vi "CIVI Read Frequency.vi"(11 "VISA Resource Name":refnum<visa-resource-name>="TCPIP0::127.0.0.1::5025::SOCKET") -> (0 "error out":errorcluster, 3 "Frequency (Hz)":i32)   [LabVIEW 2026]
panel:
  out "Raw Response":string
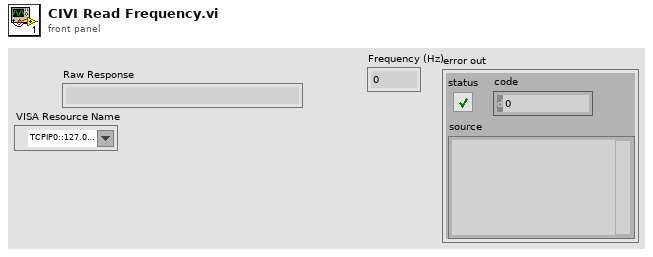
[diagram p1: front panel]
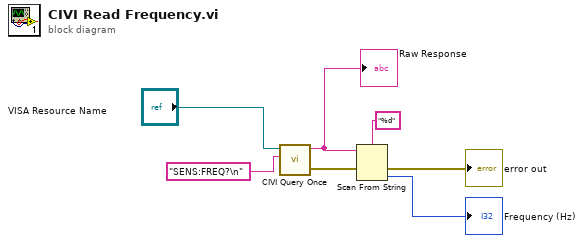
[diagram p0: block diagram]
diagram:
  n1 = call "CIVI Query Once.vi"("write buffer"="SENS:FREQ?\n", "VISA Refnum in"="VISA Resource Name") -> ("error out"=w1:errorcluster, "read buffer"=w5:string)  [unwired: 8 in]
  "Raw Response" <- w5
  n2 = Scan From String(format string="%d", input string=w5, error in=w1) -> (error out=→"error out":errorcluster, output 1=→"Frequency (Hz)":i32)  [unwired: 2 in, 2 out]
